vi "odometry_msg.vi"(11 "odometry_msg in":string) -> (1 "vel_cal":cluster{"rot_z":dbl, "lin_x":dbl}, 2 "Current_Pose":T1, 3 "robot_position_cluster":T2)   [LabVIEW 2014]
uses:
  Map_lib/MapBuilder/Robot_Position.ctl
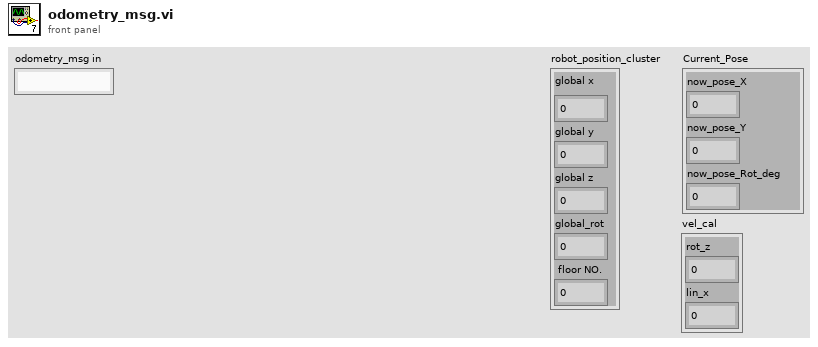
[diagram p1: front panel]
types:
  T1 = cluster{"now_pose_X":dbl, "now_pose_Y":dbl, "now_pose_Rot_deg":dbl}
  T2 = typedef "Robot_Position.ctl" = cluster{"global x":dbl, "global y":dbl, "global z":dbl, "global_rot":dbl, " floor NO.":dbl}
  T3 = cluster{"PoseCovariance":cluster{"Pose":cluster{"Point":cluster{"x":dbl, "y":dbl, "z":dbl}, "Quaternion":cluster{"x":dbl, "y":dbl, "z":dbl, "w":dbl}}, "Covariance":dbl}, "TwistCovariance":cluster{"Twist":cluster{"Linear":cluster{"x":dbl, "y":dbl, "z":dbl}, "Angular":cluster{"x":dbl, "y":dbl, "z":dbl}}, "Covariance":dbl}}
  T4 = cluster{"Roll (y)":dbl, "Pitch(x)":dbl, "Yaw (z)":dbl}
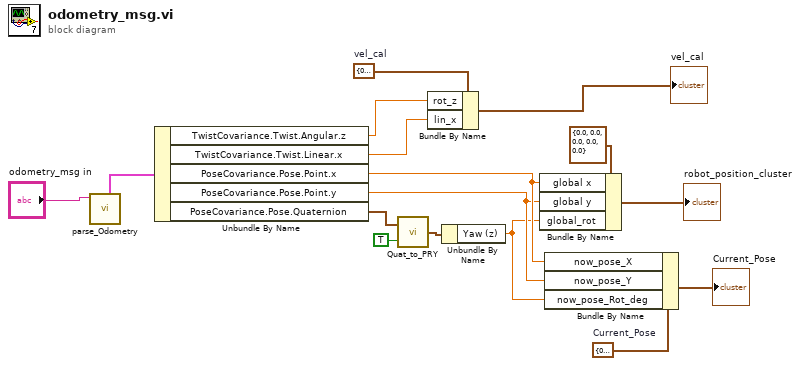
[diagram p0: block diagram]
diagram:
  w4 = cluster{"rot_z":dbl, "lin_x":dbl} {"rot_z"=0.0, "lin_x"=0.0}  # vel_cal
  w9 = T1 {"now_pose_X"=0.0, "now_pose_Y"=0.0, "now_pose_Rot_deg"=0.0}  # Current_Pose
  n1 = call <vilib>:"parse_Odometry.vi"("msg in"="odometry_msg in") -> ("Odometry"=w16:T3)  [unwired: 4 in, 4 out]
  n2 = Unbundle By Name(w16) -> ("TwistCovariance.Twist.Angular.z"=w3:dbl, "TwistCovariance.Twist.Linear.x"=w2:dbl, "PoseCovariance.Pose.Point.x"=w7:dbl, "PoseCovariance.Pose.Point.y"=w6:dbl, "PoseCovariance.Pose.Quaternion"=w15:cluster{"x":dbl, "y":dbl, "z":dbl, "w":dbl})
  n3 = call <vilib>:"Quat_to_PRY.vi"("toDegrees? (T)"=TRUE, "Quaternion"=w15) -> ("Orientation"=w13:T4)
  n4 = Bundle By Name(cluster=w4, "rot_z"=w3, "lin_x"=w2) -> (→"vel_cal":cluster{"rot_z":dbl, "lin_x":dbl})
  n5 = Unbundle By Name(w13) -> ("Yaw (z)"=w5:dbl)
  n6 = Bundle By Name(cluster=T2 {"global x"=0.0, "global y"=0.0, "global z"=0.0, "global_rot"=0.0, " floor NO."=0.0} ("robot position"), "global x"=w7, "global y"=w6, "global_rot"=w5) -> (→"robot_position_cluster":T2)
  n7 = Bundle By Name(cluster=w9, "now_pose_X"=w7, "now_pose_Y"=w6, "now_pose_Rot_deg"=w5) -> (→"Current_Pose":T1)
